vi "readValue_seqStopButton.vi"(8 "error in (no error)":errorcluster, 11 "input cluster":T1) -> (0 "error out":errorcluster, 3 "boolean value out":bool)   [LabVIEW 2021]
uses:
  TypeDefs/Tester Object.ctl
  <vilib>/NI/Modbus Library/API/Master/Modbus Master.lvclass
  <vilib>/NI/Modbus Library/API/Slave/Modbus Slave.lvclass
  Motor/Motor.lvclass
  Elevator/Elevator.lvclass
  Modbus_Master/Modbus_Master.lvclass
  ServoDrive/ServoDrive.lvclass
  TypeDefs/UIControlReferences.ctl
  TypeDefs/Devices Cluster.ctl
  Modbus/Modbus Cluster.ctl
  Modbus/Modbus Address Cluster.ctl
  DAQ/DAQNav/DAQNav Cluster.ctl
  DAQ/DAQNav/Analog Cluster.ctl
  Device Context/Device Context Cluster.ctl
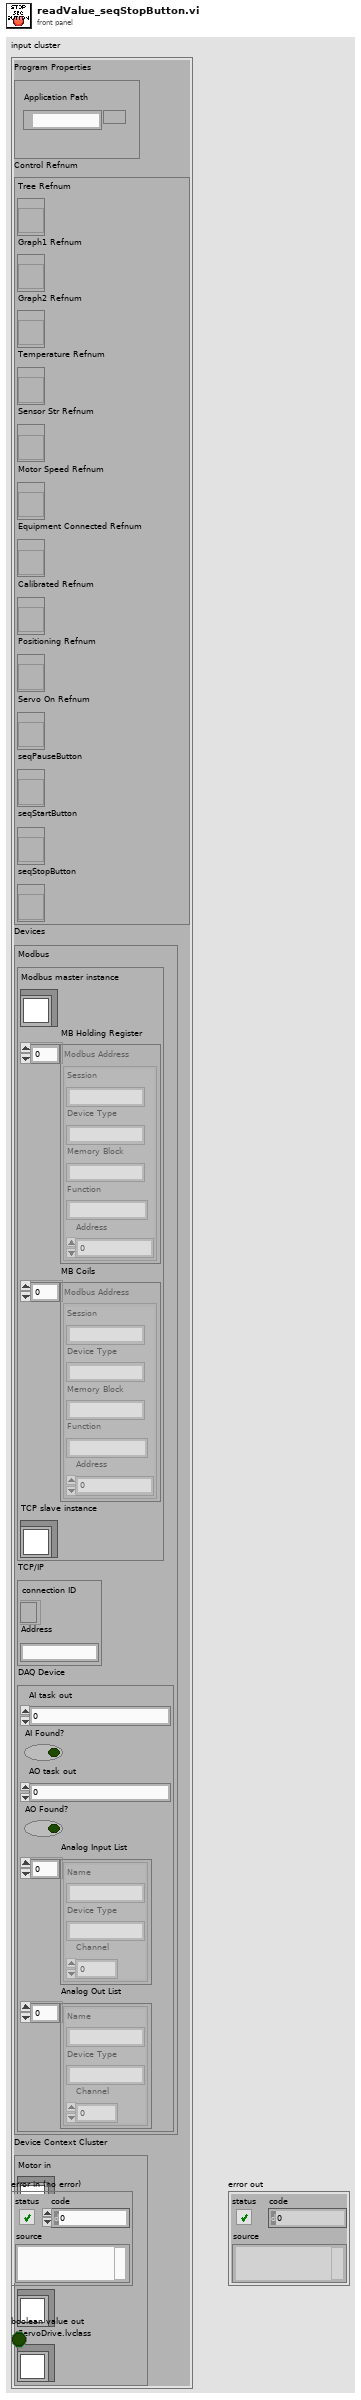
[diagram p1: front panel]
types:
  T1 = typedef "Tester Object.ctl" = cluster{"Program Properties":cluster{"Application Path":path}, "Control Refnum":T2, "Devices":T3, "Device Context Cluster":T8}
  T2 = typedef "UIControlReferences.ctl" = cluster{"Tree Refnum ":refnum<vi>, "Graph1 Refnum":refnum<vi>, "Graph2 Refnum":refnum<vi>, "Temperature Refnum":refnum<vi>, "Sensor Str Refnum":refnum<vi>, "Motor Speed Refnum":refnum<vi>, "Equipment Connected Refnum":refnum<vi>, "Calibrated Refnum":refnum<vi>, "Positioning Refnum":refnum<vi>, "Servo On Refnum":refnum<vi>, "seqPauseButton":refnum<vi>, "seqStartButton":refnum<vi>, "seqStopButton":refnum<vi>}
  T3 = typedef "Devices Cluster.ctl" = cluster{"Modbus":T4, "TCP/IP":cluster{"connection ID":refnum<k5>, "Address":string}, "DAQ Device":T6}
  T4 = typedef "Modbus Cluster.ctl" = cluster{"Modbus master instance":refnum<class "Modbus Master.lvclass">, "MB Holding Register":T5[], "MB Coils":T5[], "TCP slave instance":refnum<class "Modbus Slave.lvclass">}
  T5 = typedef "Modbus Address Cluster.ctl" = cluster{"Session":string, "Device Type":string, "Memory Block":string, "Function":string, "Address":u16}
  T6 = typedef "DAQNav Cluster.ctl" = cluster{"AI task out":i32, "AI Found?":bool, "AO task out":i32, "AO Found?":bool, "Analog Input List":T7[], "Analog Out List":T7[]}
  T7 = typedef "Analog Cluster.ctl" = cluster{"Name":string, "Device Type":string, "Channel":i32}
  T8 = typedef "Device Context Cluster.ctl" = cluster{"Motor in":refnum<class "Motor.lvclass">, "Elevator.lvclass":refnum<class "Elevator.lvclass">, "Modbus_Master.lvclass":refnum<class "Modbus_Master.lvclass">, "ServoDrive.lvclass":refnum<class "ServoDrive.lvclass">}
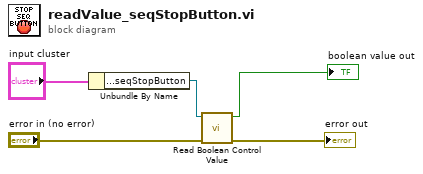
[diagram p0: block diagram]
diagram:
  n1 = Unbundle By Name("input cluster") -> ("Control Refnum.seqStopButton"=w4:refnum<vi>)
  n2 = call "Read Boolean Control Value.vi"("error in (no error)"="error in (no error)", "Boolean in"=w4) -> ("error out"=→"error out":errorcluster, "boolean value out"=→"boolean value out":bool)  [unwired: 8 in]
